vi "Ecrire config gene.vi"(2 "error in (no error)":errorcluster caption="entrée d'erreur (pas d'erreur)", 3 "refnum":T1) -> (0 "error out":errorcluster, 1 "refnum out":T1 caption="refnum en sortie")   [LabVIEW 2022 SP3]
uses:
  <vilib>/Utility/config.llb/Config Data RefNum.ctl
  Variables globales/Variable glob generale.vi
  <vilib>/Utility/config.llb/Write Key (Path).vi
  <vilib>/Utility/config.llb/Write Key (String).vi
  Variables globales/Variable glob mails.vi
  <vilib>/Utility/config.llb/NI_LVConfig.lvlib
panel:
  out "Dossier sauvegarde":path caption="Dossier sauvegarde pour enregistrement des données (il sera rempli en fonction de l'année puis du mois)"
  out "Dossier distant":path caption="Dossier distant pour enregistrement des données (il sera rempli en fonction de l'année puis du mois)"
  out "Dossier local":path caption="Dossier local pour enregistrement des données (il sera rempli en fonction de l'année puis du mois)"
  out "Nom cuve":string
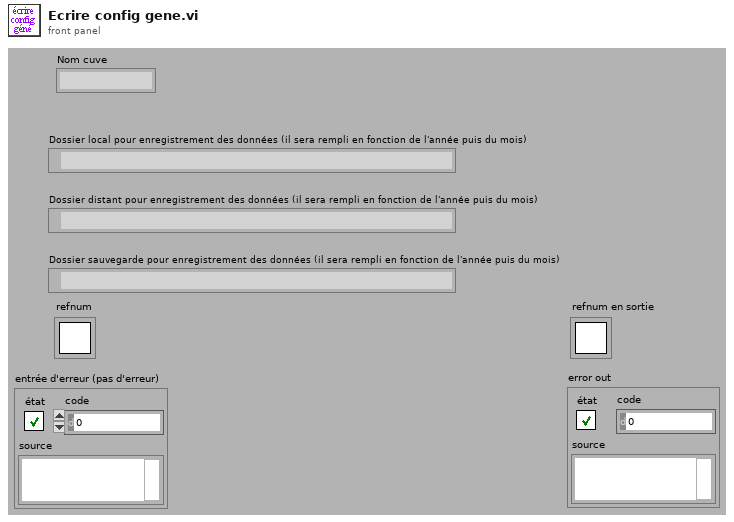
[diagram p1: front panel]
types:
  T1 = typedef "NI_LVConfig.lvlib/Config Data RefNum.ctl" = refnum<k1>
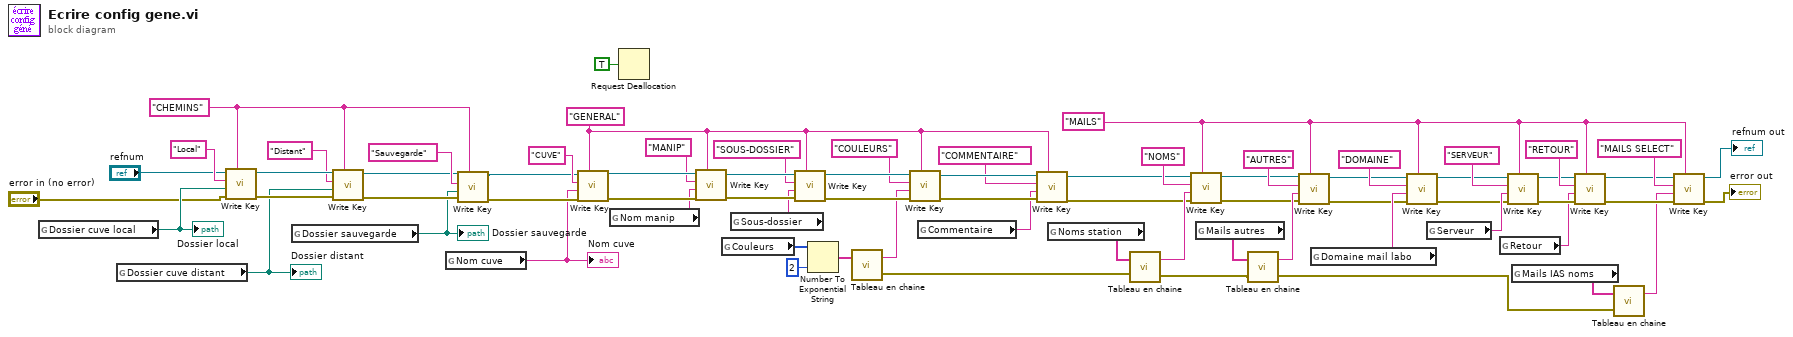
[diagram p0: block diagram]
diagram:
  w4 = "MAILS" ("section")
  w58 = "GENERAL" ("section")
  w65 = "CHEMINS" ("section")
  n1 = global read "Variable glob generale.vi" "Dossier cuve local"() -> (w62:path)
  "Dossier local" <- w62
  n2 = global read "Variable glob generale.vi" "Dossier cuve distant"() -> (w61:path)
  "Dossier distant" <- w61
  n3 = call-poly <vilib>:"Write Key.vi"("section"=w65, "error in (no error)"="error in (no error)", "value"=w62, "key"="Local", "refnum"="refnum") -> ("error out"=w69:errorcluster, "refnum out"=w70:T1)  [unwired: 4 in, 1 out]
  n4 = global read "Variable glob generale.vi" "Dossier sauvegarde"() -> (w60:path)
  "Dossier sauvegarde" <- w60
  n5 = call-poly <vilib>:"Write Key.vi"("section"=w65, "error in (no error)"=w69, "value"=w61, "key"="Distant", "refnum"=w70) -> ("error out"=w63:errorcluster, "refnum out"=w64:T1)  [unwired: 4 in, 1 out]
  n6 = global read "Variable glob generale.vi" "Nom cuve"() -> (w42:string)
  "Nom cuve" <- w42
  n7 = call-poly <vilib>:"Write Key.vi"("section"=w65, "error in (no error)"=w63, "value"=w60, "key"="Sauvegarde", "refnum"=w64) -> ("error out"=w51:errorcluster, "refnum out"=w52:T1)  [unwired: 4 in, 1 out]
  n8 = call-poly <vilib>:"Write Key.vi"("section"=w58, "error in (no error)"=w51, "value"=w42, "key"="CUVE", "refnum"=w52) -> ("error out"=w50:errorcluster, "refnum out"=w56:T1)  [unwired: 4 in, 1 out]
  n9 = global read "Variable glob generale.vi" "Nom manip"() -> (w41:string)
  n10 = Request Deallocation(TRUE ("flag")) -> ()
  n11 = call-poly <vilib>:"Write Key.vi"("section"=w58, "error in (no error)"=w50, "value"=w41, "key"="MANIP", "refnum"=w56) -> ("error out"=w49:errorcluster, "refnum out"=w54:T1)  [unwired: 4 in, 1 out]
  n12 = global read "Variable glob generale.vi" "Couleurs"() -> (w39:u32[])
  n13 = global read "Variable glob generale.vi" "Sous-dossier"() -> (w40:string)
  n14 = call-poly <vilib>:"Write Key.vi"("section"=w58, "error in (no error)"=w49, "value"=w40, "key"="SOUS-DOSSIER", "refnum"=w54) -> ("error out"=w48:errorcluster, "refnum out"=w55:T1)  [unwired: 4 in, 1 out]
  n15 = Number To Exponential String(number=w39, precision (6)=i16 2 ("précision (6)")) -> (E-format string=w37:string[])  [unwired: 2 in]
  n16 = call "Tableau en chaine.vi"("Tableau 1D"=w37) -> ("error out"=w3:errorcluster, "Chaîne"=w36:string)  [unwired: 1 in]
  n17 = call-poly <vilib>:"Write Key.vi"("section"=w58, "error in (no error)"=w48, "value"=w36, "key"="COULEURS", "refnum"=w55) -> ("error out"=w47:errorcluster, "refnum out"=w57:T1)  [unwired: 4 in, 1 out]
  n18 = global read "Variable glob generale.vi" "Commentaire"() -> (w35:string)
  n19 = call-poly <vilib>:"Write Key.vi"("section"=w58, "error in (no error)"=w47, "value"=w35, "key"="COMMENTAIRE", "refnum"=w57) -> ("error out"=w1:errorcluster, "refnum out"=w2:T1)  [unwired: 4 in, 1 out]
  n20 = global read "Variable glob mails.vi" "Noms station"() -> (w27:string[])
  n21 = call "Tableau en chaine.vi"("error in (no error)"=w3, "Tableau 1D"=w27) -> ("error out"=w11:errorcluster, "Chaîne"=w20:string)
  n22 = call-poly <vilib>:"Write Key.vi"("section"=w4, "error in (no error)"=w1, "value"=w20, "key"="NOMS", "refnum"=w2) -> ("error out"=w9:errorcluster, "refnum out"=w10:T1)  [unwired: 4 in, 1 out]
  n23 = global read "Variable glob mails.vi" "Mails autres"() -> (w26:string[])
  n24 = call "Tableau en chaine.vi"("error in (no error)"=w11, "Tableau 1D"=w26) -> ("error out"=w14:errorcluster, "Chaîne"=w19:string)
  n25 = call-poly <vilib>:"Write Key.vi"("section"=w4, "error in (no error)"=w9, "value"=w19, "key"="AUTRES", "refnum"=w10) -> ("error out"=w7:errorcluster, "refnum out"=w8:T1)  [unwired: 4 in, 1 out]
  n26 = global read "Variable glob mails.vi" "Domaine mail labo"() -> (w12:string)
  n27 = call-poly <vilib>:"Write Key.vi"("section"=w4, "error in (no error)"=w7, "value"=w12, "key"="DOMAINE", "refnum"=w8) -> ("error out"=w5:errorcluster, "refnum out"=w6:T1)  [unwired: 4 in, 1 out]
  n28 = global read "Variable glob mails.vi" "Serveur"() -> (w18:string)
  n29 = global read "Variable glob mails.vi" "Retour"() -> (w17:string)
  n30 = call-poly <vilib>:"Write Key.vi"("section"=w4, "error in (no error)"=w5, "value"=w18, "key"="SERVEUR", "refnum"=w6) -> ("error out"=w21:errorcluster, "refnum out"=w22:T1)  [unwired: 4 in, 1 out]
  n31 = global read "Variable glob mails.vi" "Mails IAS noms"() -> (w16:string[])
  n32 = call-poly <vilib>:"Write Key.vi"("section"=w4, "error in (no error)"=w21, "value"=w17, "key"="RETOUR", "refnum"=w22) -> ("error out"=w31:errorcluster, "refnum out"=w32:T1)  [unwired: 4 in, 1 out]
  n33 = call "Tableau en chaine.vi"("error in (no error)"=w14, "Tableau 1D"=w16) -> ("Chaîne"=w15:string)  [unwired: 1 out]
  n34 = call-poly <vilib>:"Write Key.vi"("section"=w4, "error in (no error)"=w31, "value"=w15, "key"="MAILS SELECT", "refnum"=w32) -> ("error out"=→"error out":errorcluster, "refnum out"=→"refnum out":T1)  [unwired: 4 in, 1 out]
